vi "Read_estimation_deletion_array_VI.vi"(10 "読み取り配列":string, 11 "元配列":string) -> (0 "逆Maxリード数":i32, 1 "逆前削減配列Max Letter X":string, 2 "順MAXリード数":i32, 3 "順前削減配列 Max L X":string, 4 "逆前削減配列判定マトリクス":bool[][](array[boolean]), 5 "読み取り長さ":i32, 6 "順前削減配列判定マトリクス":bool[][](array[boolean]), 7 "出力クラスタ":T1, 8 "重複？":bool)   [LabVIEW 2018]
panel:
  out "逆 2以上ある?":bool
  out "逆前削減 MAXL 昇順":i32[](array[numeric])
  out "逆前削減配列 Max L 昇順":string[](array[string])
  out "順 2以上ある?":bool
  out "順前削減 MAXL 昇順":i32[](array[numeric])
  out "順前削減配列 Max L 昇順":string[](array[string])
  out "逆前削減配列Max Letter マトリクス":string[](array[string])
  out "順前削減配列 Max L マトリクス":string[](array[string])
  out "逆前削減配列Max no マトリクス":i32[](array[numeric])
  out "順前削減配列Max no マトリクス":i32[](array[numeric])
  out "逆前削減配列マトリクス":string[][](array[string])
  out "順前削減配列マトリクス":string[][](array[string])
  out "逆前削減":string[](array[string])
  out "順前削減 2":string[](array[string])
  out "読み取り長さ2":i32
  # "AGAGUACA"
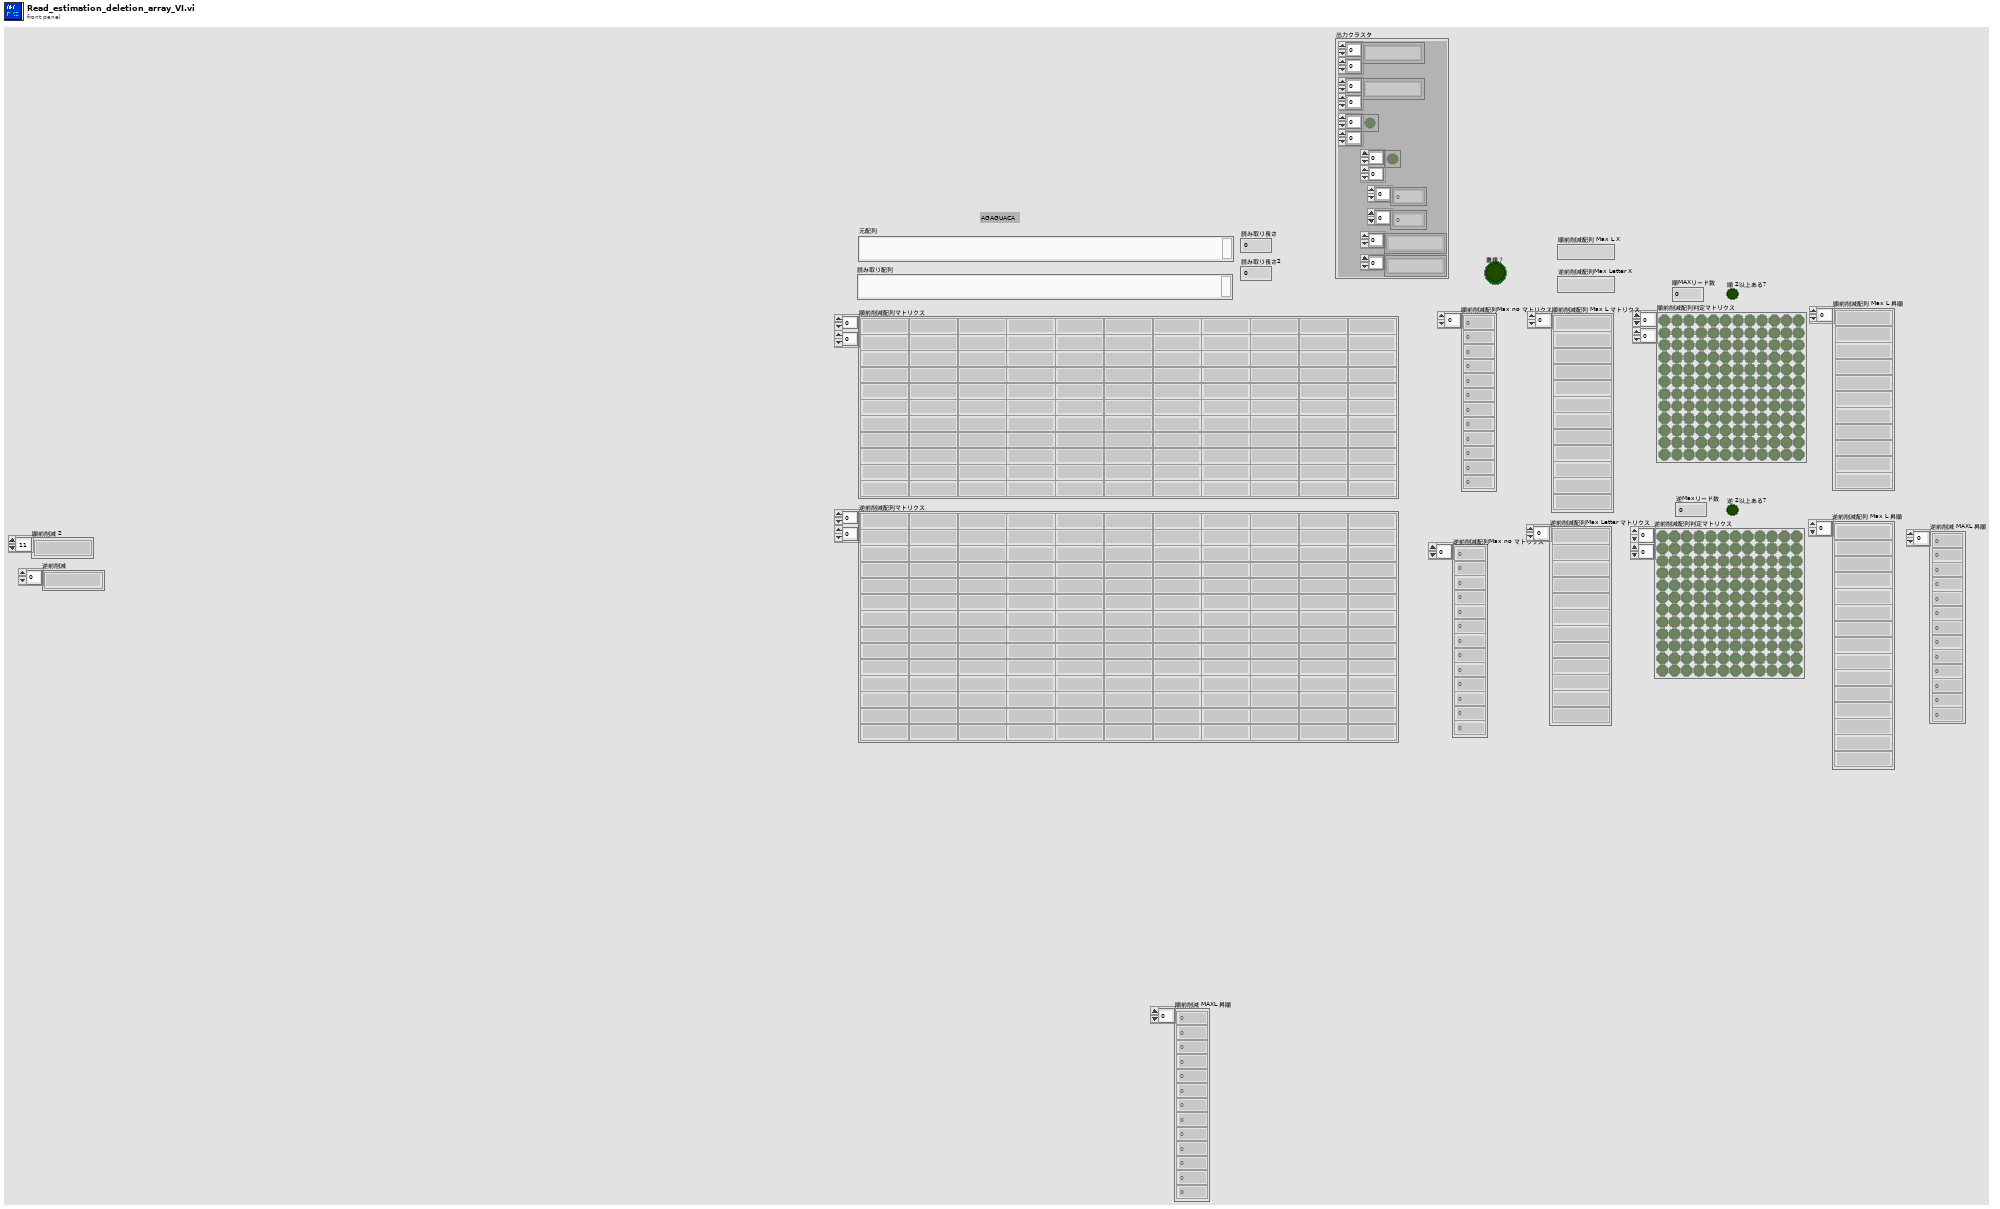
[diagram p1: front panel]
types:
  T1 = cluster{string[][], string[][], bool[][], bool[][], i32[], i32[], string[], string[]}
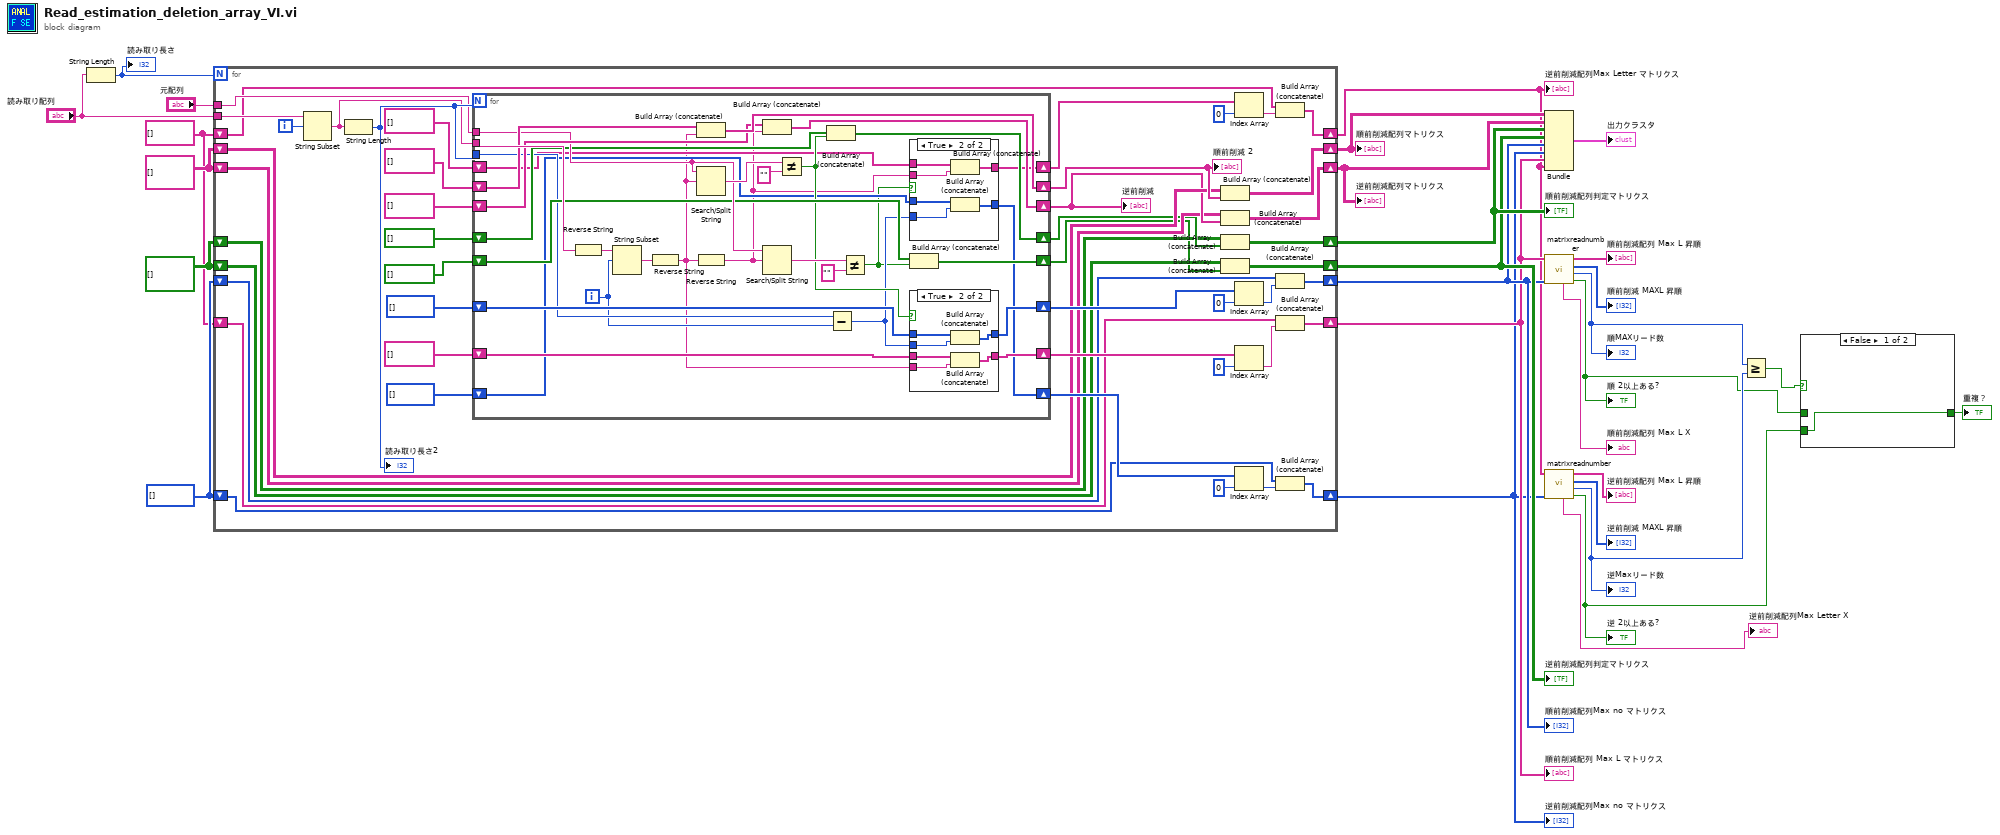
[diagram p0: block diagram]
diagram:
  w22 = string[] []
  w23 = i32[] []
  w24 = bool[][] []
  w25 = string[][] []
  n1 = String Length(string="読み取り配列") -> (length=w26:i32)
  "読み取り長さ" <- w26
  n2 = for {
    N: w26 -> [_]
    tunnel: "読み取り配列" -> [w73]
    tunnel: "元配列" -> [w54]
    shift-right: [w50] -> w21
    shift-left: w25 -> [w51]
    shift-right: [w49] -> w20
    shift-left: w25 -> [w47]
    shift-right: [w45] -> w19
    shift-left: w24 -> [w44]
    shift-right: [w43] -> w18
    shift-left: w24 -> [w42]
    shift-right: [w38] -> w11
    shift-left: w23 -> [w37]
    shift-right: [w36] -> w16
    shift-left: w23 -> [w35]
    shift-right: [w33] -> w15
    shift-left: w22 -> [w32]
    shift-right: [w31] -> w10
    shift-left: w22 -> [w29]
    i -> [w53]
    n3 = String Subset(string=w73, offset (0)=w53) -> (substring=w55:string)  [unwired: 1 in]
    n4 = String Length(string=w55) -> (length=w65:i32)
    "読み取り長さ2" <- w65
    n5 = for {
      N: w65 -> [_]
      tunnel: w55 -> [w104]
      shift-right: [w103] -> w52
      shift-left: string[] [] -> [w102]
      tunnel: w54 -> [w95]
      shift-right: [w97] -> w48
      shift-left: string[] [] -> [w96]
      shift-right: [w94] -> w41
      shift-left: bool[] [] -> [w93]
      shift-right: [w92] -> w46
      shift-left: bool[] [] -> [w91]
      shift-right: [w89] -> w57
      shift-left: string[] [] -> [w87]
      shift-right: [w86] -> w56
      shift-left: i32[] [] -> [w85]
      tunnel: w65 -> [w84]
      shift-right: [w82] -> w61
      shift-left: string[] [] -> [w81]
      shift-right: [w80] -> w60
      shift-left: i32[] [] -> [w79]
      i -> [w83]
      n6 = Reverse String(1:w104) -> (0:w75:string)
      n7 = String Subset(string=w75, offset (0)=w83) -> (substring=w88:string)  [unwired: 1 in]
      n8 = Reverse String(1:w88) -> (0:w74:string)
      n9 = Build Array (concatenate)(w102, w74) -> (w103:string[])
      n10 = Search/Split String(string=w95, search string/char (-)=w74) -> (match + rest of string=w100:string)  [unwired: 1 in, 2 out]
      n11 = Reverse String(1:w74) -> (0:w77:string)
      n12 = Build Array (concatenate)(w96, w77) -> (w97:string[])
      n13 = Search/Split String(string=w95, search string/char (-)=w77) -> (match + rest of string=w98:string)  [unwired: 1 in, 2 out]
      n14 = Not Equal?(x=w100, y="" ("ブランク")) -> (x != y?=w90:bool)
      n15 = Build Array (concatenate)(w91, w90) -> (w92:bool[])
      n16 = Subtract(x=w84, y=w83) -> (x-y=w78:i32)
      n17 = Not Equal?(x=w98, y="" ("ブランク")) -> (x != y?=w76:bool)
      n18 = case shown="True" w76 {
        tunnel: [w106 w112] -> w82
        tunnel: w77 -> [_ w111]
        tunnel: w81 -> [w106 w110]
        tunnel: [w105 w109] -> w80
        tunnel: w79 -> [w105 w108]
        tunnel: w78 -> [_ w107]
        frame False {
        }
        frame True {
          n19 = Build Array (concatenate)(w110, w111) -> (w112:string[])
          n20 = Build Array (concatenate)(w108, w107) -> (w109:i32[])
        }
      }
      n21 = Build Array (concatenate)(w93, w76) -> (w94:bool[])
      n22 = case shown="True" w90 {
        tunnel: [w114 w120] -> w89
        tunnel: w74 -> [_ w119]
        tunnel: w87 -> [w114 w118]
        tunnel: [w113 w117] -> w86
        tunnel: w85 -> [w113 w116]
        tunnel: w78 -> [_ w115]
        frame False {
        }
        frame True {
          n23 = Build Array (concatenate)(w116, w115) -> (w117:i32[])
          n24 = Build Array (concatenate)(w118, w119) -> (w120:string[])
        }
      }
    }
    "順前削減 2" <- w52
    "逆前削減" <- w48
    n25 = Build Array (concatenate)(w51, w52) -> (w50:string[][])
    n26 = Build Array (concatenate)(w47, w48) -> (w49:string[][])
    n27 = Build Array (concatenate)(w44, w46) -> (w45:bool[][])
    n28 = Build Array (concatenate)(w42, w41) -> (w43:bool[][])
    n29 = Index Array(array=w61, index=0 ("指標")) -> (element=w30:string)
    n30 = Index Array(array=w56, index=0 ("指標")) -> (element=w40:i32)
    n31 = Index Array(array=w57, index=0 ("指標")) -> (element=w34:string)
    n32 = Index Array(array=w60, index=0 ("指標")) -> (element=w39:i32)
    n33 = Build Array (concatenate)(w29, w30) -> (w31:string[])
    n34 = Build Array (concatenate)(w35, w40) -> (w36:i32[])
    n35 = Build Array (concatenate)(w32, w34) -> (w33:string[])
    n36 = Build Array (concatenate)(w37, w39) -> (w38:i32[])
  }
  "順前削減配列マトリクス" <- w21
  "逆前削減配列マトリクス" <- w20
  "順前削減配列判定マトリクス" <- w19
  "逆前削減配列判定マトリクス" <- w18
  "順前削減配列Max no マトリクス" <- w16
  "逆前削減配列Max no マトリクス" <- w11
  "順前削減配列 Max L マトリクス" <- w15
  "逆前削減配列Max Letter マトリクス" <- w10
  n37 = Bundle(w21, w20, w19, w18, w16, w11, w15, w10) -> (→"出力クラスタ":T1)  [unwired: 1 in]
  n38 = call "matrixreadnumber.vi"("順前削減配列Max no マトリクス"=w16, "順前削減配列 Max L マトリクス"=w15) -> ("2以上ある?"=w3:bool, "MAXリード数"=w6:i32, "MAXリード数昇順"=→"順前削減 MAXL 昇順":i32[], "Lリード配列昇順"=→"順前削減配列 Max L 昇順":string[], "MAXリード"=→"順前削減配列 Max L X":string)  [unwired: 5 in]
  "順 2以上ある?" <- w3
  "順MAXリード数" <- w6
  n39 = call "matrixreadnumber.vi"("順前削減配列Max no マトリクス"=w11, "順前削減配列 Max L マトリクス"=w10) -> ("2以上ある?"=w1:bool, "MAXリード数"=w5:i32, "MAXリード数昇順"=→"逆前削減 MAXL 昇順":i32[], "Lリード配列昇順"=→"逆前削減配列 Max L 昇順":string[], "MAXリード"=→"逆前削減配列Max Letter X":string)  [unwired: 5 in]
  "逆Maxリード数" <- w5
  "逆 2以上ある?" <- w1
  n40 = Greater Or Equal?(x=w6, y=w5) -> (x >= y?=w4:bool)
  n41 = case shown="False" w4 {
    tunnel: w3 -> [_ w122]
    tunnel: [w121 w122] -> w2
    tunnel: w1 -> [w121 _]
    frame False {
    }
    frame True {
    }
  }
  "重複？" <- w2
